vi "Init Msg.vi"(6 "Teller":refnum<class "Teller.lvclass">) -> (2 "Msg":refnum<class "Msg.lvclass">)   [LabVIEW 2020, in "_Template.lvlib" / "Templates.lvlib" / "TEMPLATE jettl Msg.lvlib" / "TEMPLATE.lvlib"]
uses:
  TEMPLATE.lvlib
  jettl/jettl/Teller/Teller.lvclass
  jettl/jettl/Msg/Msg.lvclass
  TEMPLATE Msg Input/TEMPLATE Msg Input/TEMPLATE Msg Input.lvclass/TEMPLATE Msg Input.ctl
  TEMPLATE Msg/TEMPLATE Msg/TEMPLATE Msg.lvclass/TEMPLATE Msg.ctl
  TEMPLATE Msg Input/TEMPLATE Msg Input/TEMPLATE Msg Input.lvclass
  C:/git/jettl/src/jettl/jettl/Msg Input/Msg Input.lvclass
  TEMPLATE Msg/TEMPLATE Msg/TEMPLATE Msg.lvclass
  C:/git/jettl/src/jettl/jettl/Msg/Msg.lvclass
  TEMPLATE Msg Input/TEMPLATE Msg Input.lvlib
  TEMPLATE Msg/TEMPLATE Msg.lvlib
panel:
  # "This front panel should not be manipulated."
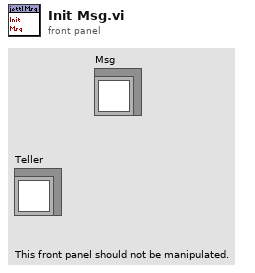
[diagram p1: front panel]
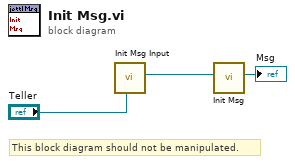
[diagram p0: block diagram]
diagram:
  # "This block diagram should not be manipulated."
  n1 = call "Init Msg Input.vi"("Teller"="Teller") -> ("Msg Input"=w3:refnum<class "Msg Input.lvclass">)  [unwired: 10 in]
  n2 = call "Init Msg.vi"("Msg Input"=w3) -> ("Msg"=→"Msg":refnum<class "Msg.lvclass">)  [unwired: 10 in]
